vi "test_simple_prompt.vi"(8 "error in":errorcluster) -> (0 "error out":errorcluster, 3 "prompt":string)   [LabVIEW 2020, in "Conformance MCP Server.lvlib"]
doc: "Conformance fixture (scenario prompts-get-simple). A prompt without arguments that returns the text \"This is a simple prompt for testing.\""
uses:
  Conformance MCP Server.lvlib
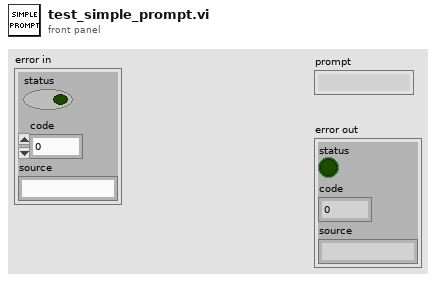
[diagram p1: front panel]
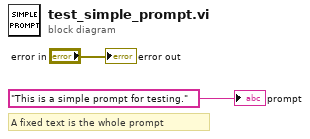
[diagram p0: block diagram]
diagram:
  # "A fixed text is the whole prompt"
  "prompt" <- "This is a simple prompt for testing." ("prompt")
  "error out" <- "error in"
